vi "GDSAPI_SetClassOptions.vi"(7 "SetAction(Set All)":T1, 8 "error in (no error)":errorcluster, 9 "WireConfiguration":T2={"Edge thickness"=1, "Edge color"=5667411, "Center thickness"=1, "Center pattern"=enum."Solid", "CenterColor1"=9740924, "CenterColor2"=8694662, "Tunnels and terminals colors"=131187}, 10 "PatternIn":T4 items=["4x4x4", "5x6x5", "6x8x6"], 11 "ProjectIconType":T5=enum."BlueFull") -> (0 "error out":errorcluster, 1 "WireConfiguration-Before":T2={"Edge thickness"=1, "Edge color"=5667411, "Center thickness"=1, "Center pattern"=enum."Solid", "CenterColor1"=9740924, "CenterColor2"=8694662, "Tunnels and terminals colors"=131187}, 2 "Pattern-Before":T4 items=["4x4x4", "5x6x5", "6x8x6"], 3 "ProjectIcon-Before":T5=enum."BlueFull")   [LabVIEW 2020]
uses:
  GDSAPI_SubVIs/GDSAPI_ProjectIconType.ctl
  ClassProviders/Common/ScriptingFunctions/Scripting_ConnectorPanePatternType.ctl
  SubVIs/GOOP_WireConfigurationType.ctl
  SubVIs/GOOP_WirePattern.ctl
  GDSAPI_SubVIs/GDSAPI_SetClassOptionsAction.ctl
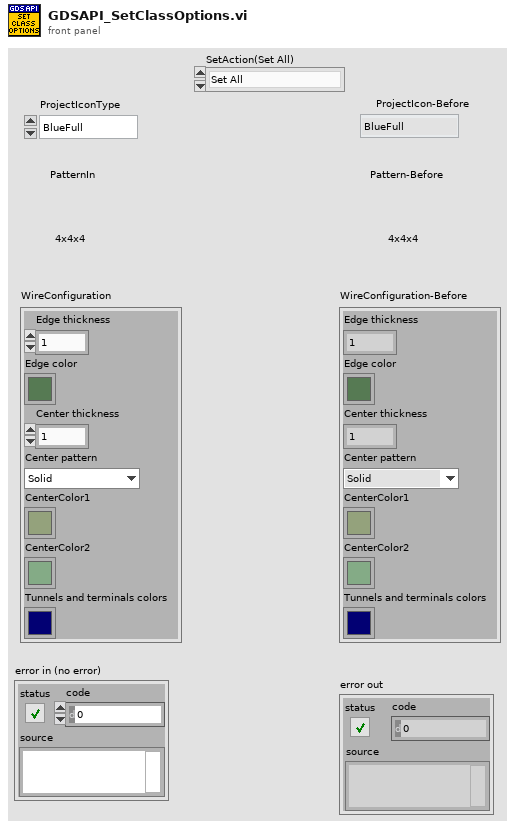
[diagram p1: front panel]
types:
  T1 = typedef "GDSAPI_SetClassOptionsAction.ctl" = enum16{"Set All", "Set Project Icon Type", "Set Pattern Type", "Set Wire Configuration"}
  T2 = typedef "GOOP_WireConfigurationType.ctl" = cluster{"Edge thickness":i32, "Edge color":u32, "Center thickness":i32, "Center pattern":T3, "CenterColor1":u32, "CenterColor2":u32, "Tunnels and terminals colors":u32}
  T3 = typedef "GOOP_WirePattern.ctl" = enum16{"Solid", "Large dash", "Small dash"}
  T4 = typedef "Scripting_ConnectorPanePatternType.ctl" = u16
  T5 = typedef "GDSAPI_ProjectIconType.ctl" = enum16{"BlueCircle", "BlueFrame", "BlueFull", "BlueMessage", "BrownCircle", "BrownFrame", "BrownFull", "BurgundyCircle", "BurgundyFrame", "BurgundyFull", "CyanCircle", "CyanFrame", "CyanFull", "DarkBlueCircle", "DarkBlueFrame", "DarkBlueFull", "ForestGreenCircle", "ForestGreenFrame", "ForestGreenFull", "GrayCircle", "GrayFrame", "GrayFull", "GreenCircle", "GreenFrame", "GreenFull", "Interface", "InterfaceBlue", "InterfaceBrown", "InterfaceBurgundy", "InterfaceCyan", "InterfaceDarkBlue", "InterfaceForestGreen", "InterfaceGray", "InterfaceGreen", "InterfaceLightGreen", "InterfaceLightRed", "InterfacePink", "InterfacePurple", "InterfaceRed", "InterfaceYellow", "LightGreenCircle", "LightGreenFrame", "LightGreenFull", "LightRedCircle", "LightRedFrame", "LightRedFull", "PinkCircle", "PinkFrame", "PinkFull", "PurpleCircle", "PurpleFrame", "PurpleFull", "RedCircle", "RedFrame", "RedFull", "YellowCircle", "YellowFrame", "YellowFull"}
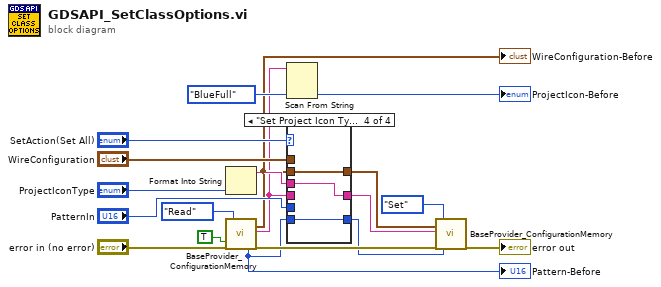
[diagram p0: block diagram]
diagram:
  n1 = Format Into String("ProjectIconType") -> (resulting string=w8:string)  [unwired: 3 in, 1 out]
  n2 = call "BaseProvider_ConfigurationMemory.vi"("Filter_Icons"=TRUE, "error in (no error)"="error in (no error)", "Action"=enum16{"Read", "Load", "Save", "Set"}."Read") -> ("PatternOut"=w2:T4, "WireConfigurationOut"=w3:T2, "IconOut"=w1:string, "error out"=w14:errorcluster)  [unwired: 10 in, 3 out]
  "Pattern-Before" <- w2
  "WireConfiguration-Before" <- w3
  n3 = Scan From String(input string=w1, default 1=GDSAPI_ProjectIconType."BlueFull" ("ProjectIcon-Before")) -> (output 1=→"ProjectIcon-Before":T5)  [unwired: 3 in, 3 out]
  n4 = case shown="\"Set Project Icon Type\"" "SetAction(Set All)" {
    tunnel: "WireConfiguration" -> [w22 _ w27 _]
    tunnel: w8 -> [w21 _ _ w30]
    tunnel: "PatternIn" -> [w20 w25 _ _]
    tunnel: [w22 w24 w27 w31] -> w6
    tunnel: [w21 w23 w28 w30] -> w5
    tunnel: [w20 w25 w26 w29] -> w4
    tunnel: w3 -> [_ w24 _ w31]
    tunnel: w2 -> [_ _ w26 w29]
    tunnel: w1 -> [_ w23 w28 _]
    frame "Set All", Default {
    }
    frame "Set Pattern Type" {
    }
    frame "Set Wire Configuration" {
    }
    frame "Set Project Icon Type" {
    }
  }
  n5 = call "BaseProvider_ConfigurationMemory.vi"("WireConfiguration"=w6, "Icon"=w5, "error in (no error)"=w14, "Action"=enum16{"Read", "Load", "Save", "Set"}."Set", "PatternIn"=w4) -> ("error out"=→"error out":errorcluster)  [unwired: 8 in, 6 out]
